vi "Deposit Amount.vi"(0 "Amount":dbl, 5 "Session in":T1, 11 "error in":errorcluster) -> (4 "Session out":T1, 15 "error out":errorcluster)   [LabVIEW 2026, in "ATM.lvlib"]
doc: "Deposits Amount into the session's account through the Account Manager module (Deposit request, which updates the accounts file) and shows the Deposit Complete message with the TRANSACTION amount. Nothing is pending afterwards."
uses:
  ATM.lvlib
  Libraries/Account Manager/Account Manager.lvlib
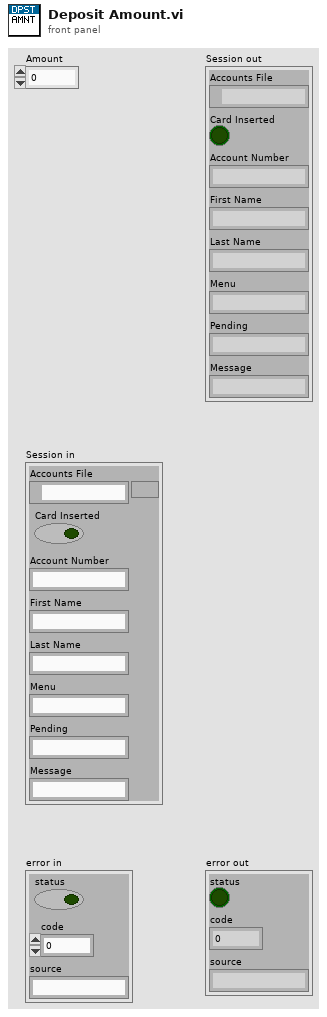
[diagram p1: front panel]
types:
  T1 = cluster{"Accounts File":path, "Card Inserted":bool, "Account Number":string, "First Name":string, "Last Name":string, "Menu":string, "Pending":string, "Message":string}
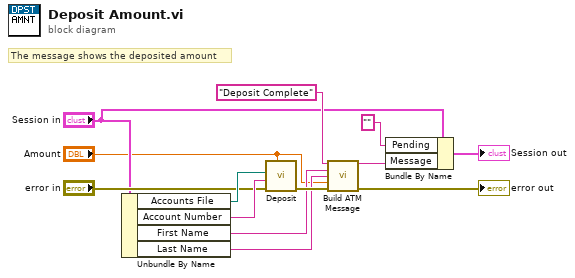
[diagram p0: block diagram]
diagram:
  # "The message shows the deposited amount"
  n1 = Unbundle By Name("Session in") -> ("Accounts File"=w4:path, "Account Number"=w5:string, "First Name"=w6:string, "Last Name"=w7:string)
  n2 = call "Deposit.vi"("Amount"="Amount", "error in"="error in", "Account Number"=w5, "Accounts File"=w4) -> ("error out"=w8:errorcluster)  [unwired: 5 in, 2 out]
  n3 = call "Build ATM Message.vi"("Message Name"="Deposit Complete", "First Name"=w6, "Last Name"=w7, "Amount"="Amount", "error in"=w8) -> ("Message"=w10:string, "error out"=→"error out":errorcluster)  [unwired: 9 in]
  n4 = Bundle By Name(cluster="Session in", "Pending"="" ("nothing pending"), "Message"=w10) -> (→"Session out":T1)
